vi "Linear-spline ramp.vi"(9 "Total Samples":i32, 10 "Ramp Samples":i32) -> (2 "Ramp pattern":dbl[](array[numeric]))   [LabVIEW 2020, in "Scan Generators.lvlib"]
uses:
  <vilib>/Analysis/1siggen.llb/Ramp Pattern by Samples.vi
  <vilib>/Analysis/1siggen.llb/Ramp Pattern by Delta.vi
  Scan Generators.lvlib
  <vilib>/gmath/NI_Gmath.lvlib
  <vilib>/Analysis/NI_AALBase.lvlib
panel:
  out "Waveform Graph":dbl[](graph)
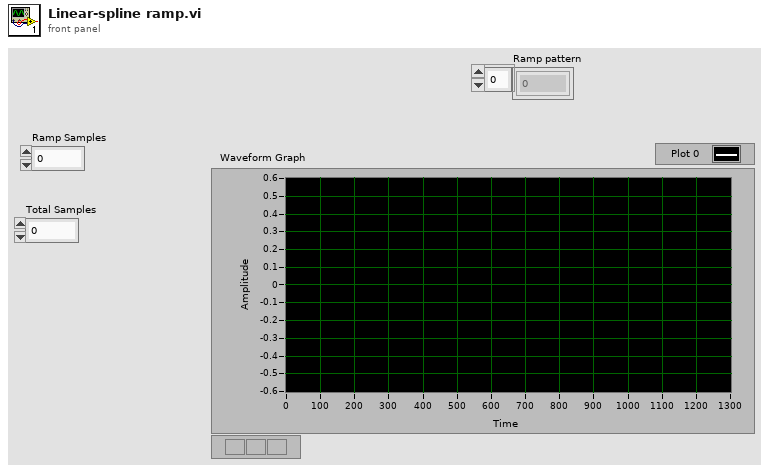
[diagram p1: front panel]
types:
  T1 = cluster{"boundary":enum16{"natural spline", "not-a-knot", "1st derivative", "2nd derivative"}, "derivative value":dbl}
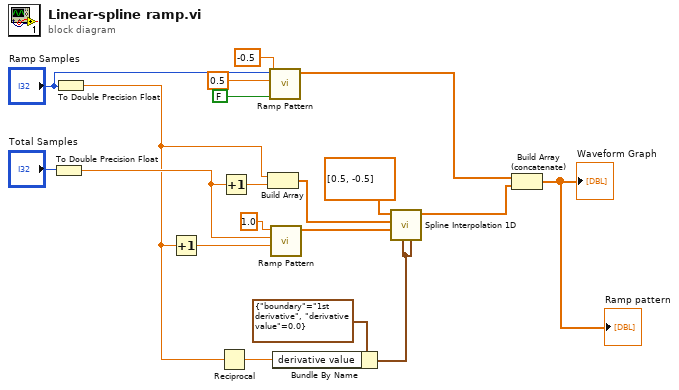
[diagram p0: block diagram]
diagram:
  n1 = To Double Precision Float(number="Total Samples") -> (double precision float=w11:dbl)
  n2 = To Double Precision Float(number="Ramp Samples") -> (double precision float=w10:dbl)
  n3 = Increment(x=w10) -> (x+1=w9:dbl)
  n4 = Reciprocal(x=w10) -> (1/x=w18:dbl)
  n5 = Increment(x=w11) -> (x+1=w12:dbl)
  n6 = Build Array(w10, w12) -> (w8:dbl[])
  n7 = call-poly <vilib>:"Ramp Pattern.vi"("exclude end?"=FALSE, "start"=-0.5, "end"=0.5, "samples"="Ramp Samples") -> ("Ramp Pattern"=w3:dbl[])  [unwired: 6 in, 1 out]
  n8 = call-poly <vilib>:"Ramp Pattern.vi"("start"=w9, "end"=w11, "delta"=1.0) -> ("Ramp Pattern"=w15:dbl[])  [unwired: 6 in, 2 out]
  n9 = Bundle By Name(cluster=T1 {"boundary"=enum."1st derivative", "derivative value"=0.0} ("initial boundary"), "derivative value"=w18) -> (w17:T1)
  n10 = call <vilib>:"Spline Interpolation 1D.vi"("final boundary"=w17, "initial boundary"=w17, "xi"=w15, "X"=w8, "Y"=dbl[] [0.5, -0.5]) -> ("yi"=w7:dbl[])  [unwired: 4 in, 2 out]
  n11 = Build Array (concatenate)(w3, w7) -> (→"Waveform Graph" →"Ramp pattern":dbl[])
